vi "FuncVI-SndOut.vi"(5 "InstanceRef":T2, 9 "arg list":T1[](array[typedef]) {"num" format="%.2f"}) -> (0 "error out":bool, 3 "result":T1 {"num" format="%.2f"})   [LabVIEW 2021]
doc: "<B>FuncVI-SndOut</B>\n\nThis VI is example of implementation of CalcExpress function (FuncVI). The function writes sound represented as 1D Array of DBL values to a sound output device.\n\n::: CalcExpress Toolkit :::\nCopyright (c) 2000-2026 Konstantin Shifershteyn. All rights reserved."
uses:
  vi.lib/addons/CalcExpress/cetypes.llb/CalcExpress Function Argument Info.ctl
  vi.lib/addons/CalcExpress/cetypes.llb/CalcExpress Instance RefNum.ctl
  <vilib>/sound2/lvsound2.llb/Sound Data Format.ctl
  <vilib>/sound2/lvsound2.llb/Sampling Mode.ctl
  <vilib>/sound2/lvsound2.llb/Sound Output Write (DBL Single).vi
panel:
  in  "max arg num":i32=3
  in  "min arg num":i32=3
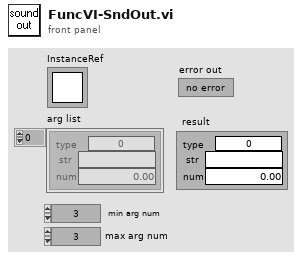
[diagram p1: front panel]
types:
  T1 = typedef "CalcExpress Function Argument Info.ctl" = cluster{"type":u32, "str":string, "num":dbl}
  T2 = typedef "CalcExpress Instance RefNum.ctl" = refnum<k1>
  T3 = enum32{"String", "DBL Number", "identifier", "1D Array of DBL", "2D Array of DBL", "CDB Number", "1D Array of CDB", "2D Array of CDB", "1D Array of String", "2D Array of String", "Unknown data type"}
  T4 = cluster{"index":i32, "data type":enum32{"String", "DBL Number", "identifier", "1D Array of DBL", "2D Array of DBL", "CDB Number", "1D Array of CDB", "2D Array of CDB", "1D Array of String", "2D Array of String", "Unknown data type"}, "default num":dbl, "default str":string}[]
  T5 = typedef "Sound Data Format.ctl" = cluster{"sample rate (S/s)":dbl, "number of channels":i32, "bits per sample":i32}
  T6 = typedef "Sampling Mode.ctl" = i32
  T7 = typedef "Sound Output Task ID.ctl" = u32
  T8 = cluster{"data type":enum32{"String", "DBL Number", "identifier", "1D Array of DBL", "2D Array of DBL", "CDB Number", "1D Array of CDB", "2D Array of CDB", "1D Array of String", "2D Array of String", "Unknown data type"}, string, dbl}
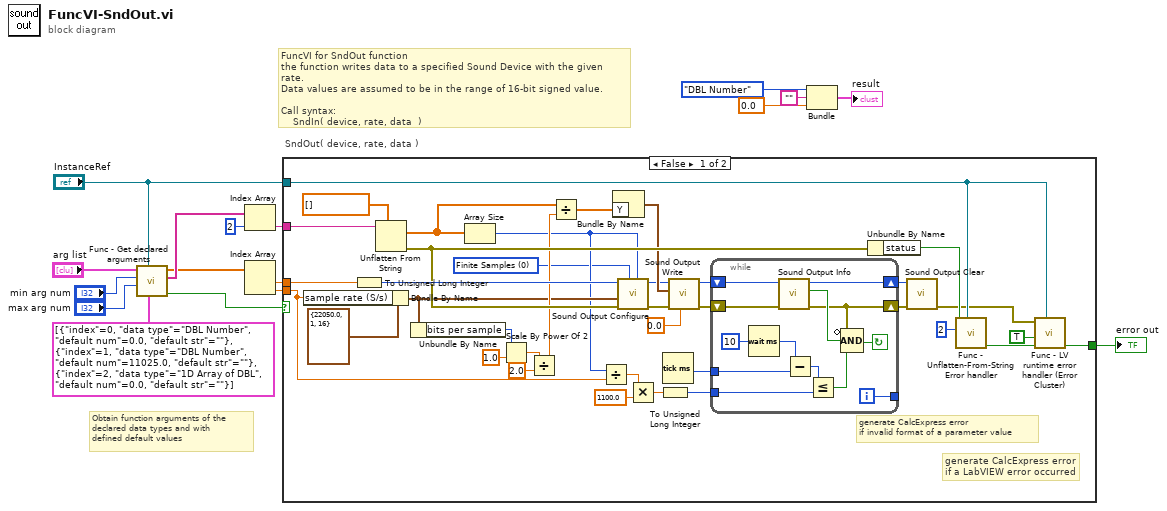
[diagram p0: block diagram]
diagram:
  # "FuncVI for SndOut function\nthe function writes data to a specified Sound Device with the given rate.\nData values are assumed to be in the range of 16-bit signed value.\n\nCall syntax:\n    SndIn( device, rate, data  )"
  # "Obtain function arguments of the\ndeclared data types and with\ndefined default values"
  # "SndOut( device, rate, data )"
  n1 = call "Func - Get declared arguments.vi"("arg descriptors"=T4 [{"index"=0, "data type"=enum."DBL Number", "default num"=0.0, "default str"=""}, {"index"=1, "data type"=enum."DBL Number", "default num"=11025.0, "default str"=""}, {"index"=2, "data type"=enum."1D Array of DBL", "default num"=0.0, "default str"=""}] ("args descriptors"), "InstanceRef"="InstanceRef", "max arg num"="max arg num", "min arg num"="min arg num", "arg list"="arg list") -> ("error out"=w15:bool, "str list"=w10:string[], "num list"=w1:dbl[])  [unwired: 3 in, 1 out]
  n2 = Index Array(array=w10, index=2) -> (element=w9:string)
  n3 = Index Array(array=w1) -> (element #1=w3:dbl, element #2=w2:dbl)  [unwired: 2 in]
  n4 = case shown="False" w15 {
    selector: w15 -> [_ w68]
    tunnel: [w51 w68] -> w14
    tunnel: "InstanceRef" -> [w48 _]
    tunnel: w2 -> [w22 _]
    tunnel: w3 -> [w52 _]
    tunnel: w9 -> [w54 _]
    frame False {
      w21 = T6 0 items=["Finite Samples", "Continuous Samples"] ("sample mode")
      # "generate CalcExpress error\nif invalid format of a parameter value"
      # "generate CalcExpress error\nif a LabVIEW error occurred"
      n5 = Bundle By Name(cluster=T5 {"sample rate (S/s)"=22050.0, "number of channels"=1, "bits per sample"=16} ("sound format"), "sample rate (S/s)"=w22) -> (w35:T5)
      n6 = To Unsigned Long Integer(number=w52) -> (unsigned 32bit integer=w43:u32)
      n7 = Unflatten From String(type=dbl[] [] ("double precision float"), binary string=w54) -> (value=w26:dbl[], error out=w42:errorcluster)  [unwired: 3 in, 1 out]
      n8 = Unbundle By Name(w35) -> ("bits per sample"=w40:i32)
      n9 = Array Size(array=w26) -> (size(s)=w23:i32)
      n10 = Scale By Power Of 2(n=w40, x=1.0) -> (x*2^n=w38:dbl)
      n11 = Divide(x=w38, y=2.0) -> (x/y=w36:dbl)
      n12 = Divide(x=w26, y=w36) -> (x/y=w32:dbl[])
      n13 = Divide(x=w23, y=w22) -> (x/y=w25:dbl)
      n14 = Bundle By Name("Y"=w32) -> (w41:waveform(dbl))  [unwired: 1 in]
      n15 = call <vilib>:"Sound Output Configure.vi"("number of samples/ch"=w23, "sample mode"=w21, "error in (no error)"=w42, "sound format"=w35, "device ID"=w43) -> ("error out"=w33:errorcluster, "task ID"=w34:T7)  [unwired: 5 in]
      n16 = Multiply(x=w25, y=1100.0) -> (x*y=w20:dbl)
      n17 = To Unsigned Long Integer(number=w20) -> (unsigned 32bit integer=w19:u32)
      n18 = Tick Count (ms)() -> (millisecond timer value=w27:u32)
      n19 = call-poly <vilib>:"Sound Output Write.vi"("timeout (sec)"=0.0, "error in (no error)"=w33, "data"=w41, "task ID"=w34) -> ("error out"=w30:errorcluster, "task ID out"=w31:T7)  [unwired: 6 in]
      n20 = while {
        shift-right: [w65] -> w28
        shift-left: w31 -> [w67]
        shift-right: [w56] -> w29
        shift-left: w30 -> [w66]
        tunnel: w27 -> [w61]
        tunnel: w19 -> [w58]
        tunnel: [w57] -> _
        i -> [w57]
        stop <- w55 continue-if-true
        n21 = Wait (ms)(milliseconds to wait=u32 10) -> (millisecond timer value=w62:u32)
        n22 = call <vilib>:"Sound Output Info.vi"("error in (no error)"=w66, "task ID"=w67) -> ("error out"=w56:errorcluster, "is playing?"=w64:bool, "task ID out"=w65:T7)  [unwired: 6 in, 1 out]
        n23 = Subtract(x=w62, y=w61) -> (x-y=w60:u32)
        n24 = Less Or Equal?(x=w60, y=w58) -> (x <= y?=w59:bool)
        n25 = Compound Arithmetic op=AND(invert w56, w64, w59) -> (w55:bool)
      }
      n26 = Unbundle By Name(w42) -> ("status"=w49:bool)
      n27 = call <vilib>:"Sound Output Clear.vi"("error in (no error)"=w29, "task ID"=w28) -> ("error out"=w44:errorcluster)  [unwired: 9 in]
      n28 = call "Func - Unflatten-From-String Error handler.vi"("InstanceRef"=w48, "argument number"=2, "Unflatten Error status"=w49) -> ("error out"=w46:bool)  [unwired: 6 in]
      n29 = call "Func - LV runtime error handler (Error Cluster).vi"("InstanceRef"=w48, "error in"=w46, "Gen CE error?"=TRUE, "LabVIEW error"=w44) -> ("error out"=w51:bool)  [unwired: 2 in, 3 out]
    }
    frame True {
    }
  }
  "error out" <- w14
  n30 = Bundle("data type"=T3."DBL Number", "", 0.0) -> (→"result":T8)  [unwired: 1 in]
